vi "voxelization.vi"(8 "격자크기":dbl=20.0, 10 "Y":dbl[](array[numeric]), 11 "X":dbl[](array[numeric])) -> (2 "voxeled_y":i32[](array[numeric]), 3 "voxeled_x":i32[](array[numeric]))   [LabVIEW 2024]
uses:
  f0a341ce-9988-40be-8e37-12ecbde367e4.vi
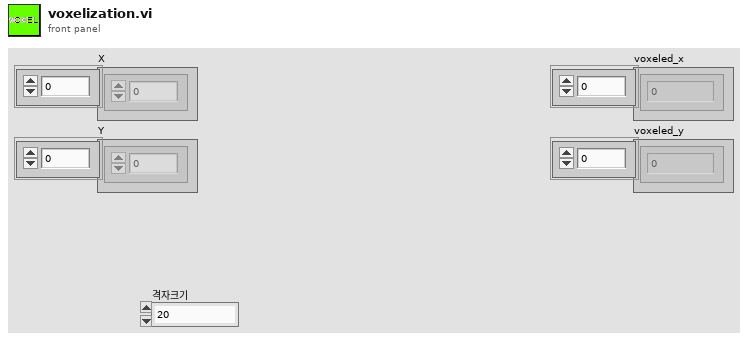
[diagram p1: front panel]
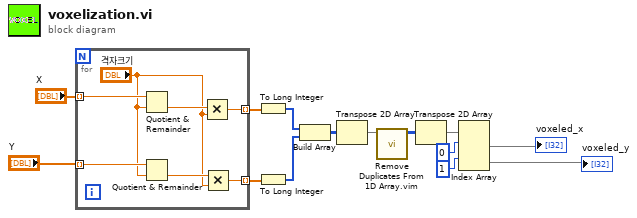
[diagram p0: block diagram]
diagram:
  n1 = for {
    tunnel: "X" -> [w21] mode=indexing
    tunnel: "Y" -> [w20] mode=indexing
    tunnel: [w17] -> w8 mode=indexing
    tunnel: [w16] -> w7 mode=indexing
    n2 = Quotient & Remainder(x=w21, y="격자크기") -> (floor(x/y)=w19:dbl)  [unwired: 1 out]
    n3 = Quotient & Remainder(x=w20, y="격자크기") -> (floor(x/y)=w18:dbl)  [unwired: 1 out]
    n4 = Multiply(x=w19, y="격자크기") -> (x*y=w17:dbl)
    n5 = Multiply(x=w18, y="격자크기") -> (x*y=w16:dbl)
  }
  n6 = To Long Integer(number=w8) -> (32bit integer=w11:i32[])
  n7 = To Long Integer(number=w7) -> (32bit integer=w12:i32[])
  n8 = Build Array(w11, w12) -> (w10:i32[][])
  n9 = Transpose 2D Array(2D array=w10) -> (transposed array=w14:i32[][])
  n10 = call "Remove Duplicates From 1D Array.vim"("array"=w14) -> ("array with duplicates removed"=w13:i32[][])  [unwired: 10 in]
  n11 = Transpose 2D Array(2D array=w13) -> (transposed array=w9:i32[][])
  n12 = Index Array(array=w9, index (row) #1=0 ("index (row)"), index (row) #2=1 ("index (row)")) -> (element #1=→"voxeled_x":i32[], element #2=→"voxeled_y":i32[])  [unwired: 2 in]
